vi "PicoScope5000aSettings.vi"(0 "error in":errorcluster, 1 "Channel A Settings":T3={"Enabled"=FALSE, "Coupling"=1, "Range"=6, "Analogue Offset"=0.0, "Bandwidth Limit"=0} {"Bandwidth Limit" items=["Full", "20MHz"]; "Range" items=["10 mV", "20 mV", "50 mV", "100 mV", "200 mV", "500 mV", "1 V", "2 V", "5 V", "10 V", "20 V"]; "Coupling" items=["AC", "DC"]}, 2 "Port 0 Settings":T1={"Enabled"=FALSE, "Logic Level"=9830} {"Logic Level" items=["1.5V TTL"=9830, "2.5V CMOS"=16383]}, 3 "Channel B Settings":T3={"Enabled"=FALSE, "Coupling"=1, "Range"=6, "Analogue Offset"=0.0, "Bandwidth Limit"=0} {"Bandwidth Limit" items=["Full", "20MHz"]; "Range" items=["10 mV", "20 mV", "50 mV", "100 mV", "200 mV", "500 mV", "1 V", "2 V", "5 V", "10 V", "20 V"]; "Coupling" items=["AC", "DC"]}, 5 "handle in":i16, 9 "Device Info":T2, 11 "Trigger Settings":T4={"Trigger Enabled"=FALSE, "Trigger Source"=enum."Channel A", "Trigger Threshold (volts)"=0.0, "Trigger Direction"=2, "Trigger Delay (samples)"=0, "Auto Trigger Time (ms)"=1000} {"Trigger Direction" items=["Rising"=2, "Falling"=3]}, 12 "Channel C Settings":T3={"Enabled"=FALSE, "Coupling"=1, "Range"=6, "Analogue Offset"=0.0, "Bandwidth Limit"=0} {"Bandwidth Limit" items=["Full", "20MHz"]; "Range" items=["10 mV", "20 mV", "50 mV", "100 mV", "200 mV", "500 mV", "1 V", "2 V", "5 V", "10 V", "20 V"]; "Coupling" items=["AC", "DC"]}, 13 "Port 1 Settings":T1={"Enabled"=FALSE, "Logic Level"=9830} {"Logic Level" items=["1.5V TTL"=9830, "2.5V CMOS"=16383]}, 14 "Channel D Settings":T3={"Enabled"=FALSE, "Coupling"=1, "Range"=6, "Analogue Offset"=0.0, "Bandwidth Limit"=0} {"Bandwidth Limit" items=["Full", "20MHz"]; "Range" items=["10 mV", "20 mV", "50 mV", "100 mV", "200 mV", "500 mV", "1 V", "2 V", "5 V", "10 V", "20 V"]; "Coupling" items=["AC", "DC"]}, 15 "Max ADC value":i16) -> (4 "error out":errorcluster, 6 "handle out":i16, 8 "enabled array":i16[](array[numeric]))   [LabVIEW 2010]
doc: "This VI is used to set up the oscilloscope. The inputs are clusters for setting channel and simple trigger settings. Advanced triggers can be set up using PicoScope3000aAdvancedTriggerSettings.vi"
uses:
  ps5000a.dll
  PicoScope5000aAnalogChannelSettings.ctl
  PicoScope5000aDigitalChannelSettings.ctl
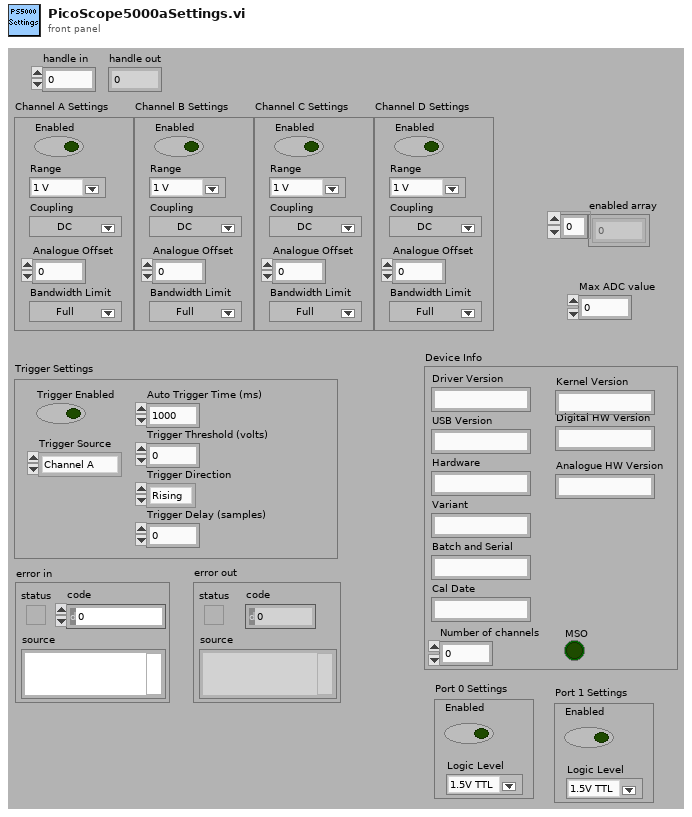
[diagram p1: front panel]
types:
  T1 = typedef "PicoScope5000aDigitalChannelSettings.ctl" = cluster{"Enabled":bool, "Logic Level":i16}
  T2 = cluster{"Driver Version":string, "USB Version":string, "Hardware":string, "Variant":string, "Batch and Serial":string, "Cal Date":string, "Kernel Version":string, "Digital HW Version":string, "Analogue HW Version":string, "MSO":bool, "Number of channels":i16}
  T3 = typedef "PicoScope5000aAnalogChannelSettings.ctl" = cluster{"Enabled":bool, "Coupling":i16, "Range":u16, "Analogue Offset":sgl, "Bandwidth Limit":u32}
  T4 = cluster{"Trigger Enabled":bool, "Trigger Source":enum16{"Channel A", "Channel B", "Channel C", "Channel D", "Ext."}, "Trigger Threshold (volts)":dbl, "Trigger Direction":u16, "Trigger Delay (samples)":u32, "Auto Trigger Time (ms)":i16}
  T5 = enum16{"Channel A", "Channel B", "Channel C", "Channel D", "Ext."}
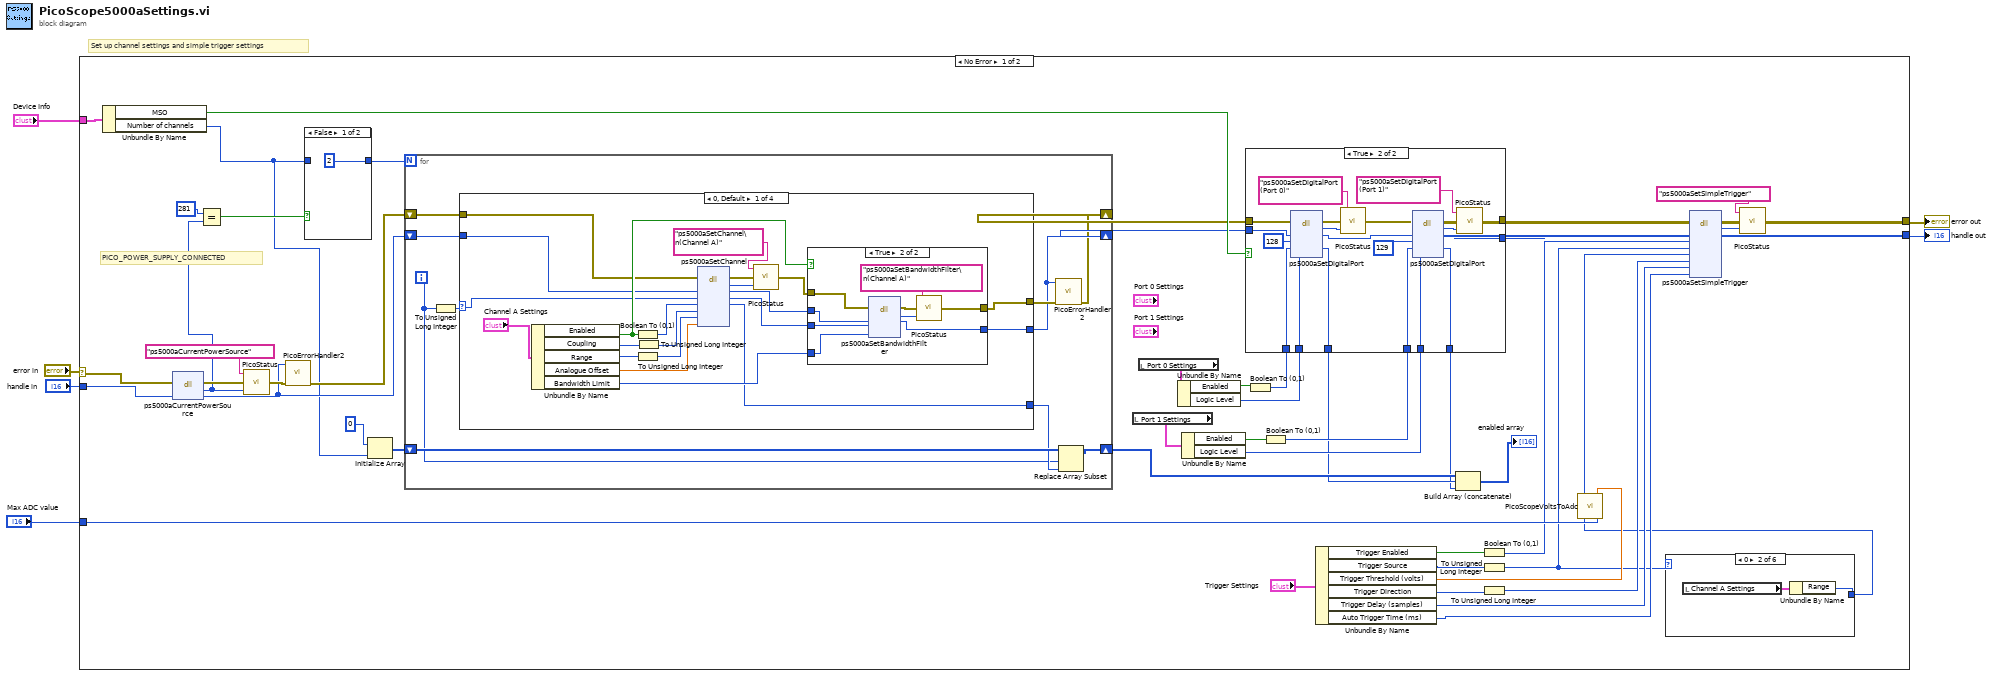
[diagram p0: block diagram]
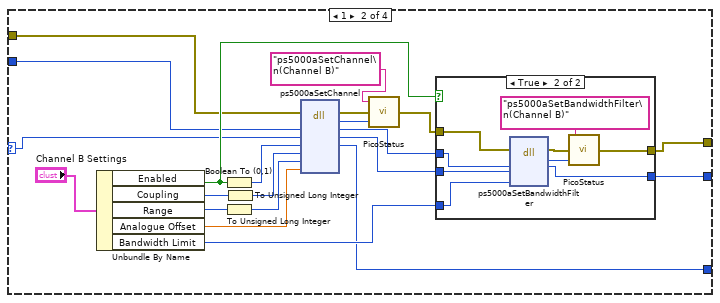
[diagram p4: hidden frame]
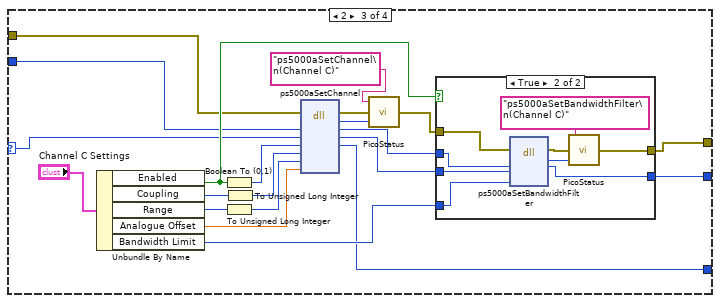
[diagram p6: hidden frame]
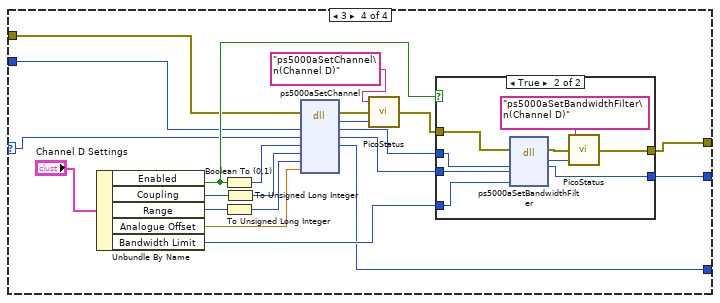
[diagram p8: hidden frame]
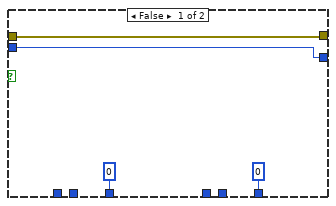
[diagram p10: hidden frame]
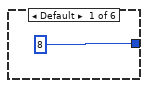
[diagram p11: hidden frame]
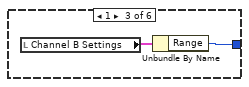
[diagram p12: hidden frame]
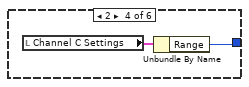
[diagram p13: hidden frame]
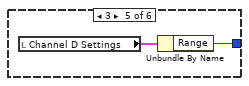
[diagram p14: hidden frame]
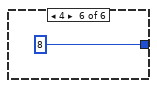
[diagram p15: hidden frame]
diagram:
  # "Set up channel settings and simple trigger settings"
  n1 = case shown="No Error" "error in" {
    selector: "error in" -> [w19 w232]
    tunnel: "handle in" -> [w18 w231]
    tunnel: [w47 w231] -> w4
    tunnel: [w36 w232] -> w3
    tunnel: "Device Info" -> [w42 _]
    tunnel: "Max ADC value" -> [w39 _]
    frame No Error {
      # "PICO_POWER_SUPPLY_CONNECTED"
      n2 = Unbundle By Name(w42) -> ("MSO"=w24:bool, "Number of channels"=w7:i16)
      n3 = dll-call lib="ps5000a.dll" fn="ps5000aCurrentPowerSource"(error in=w19, "handle"=w18) -> (error out=w45:errorcluster, "PICO_STATUS"=w43:u32, "handle"=w16:i16)  [unwired: 2 in, 1 out]
      n4 = Equal?(x=u32 281, y=w43) -> (x = y?=w14:bool)
      n5 = call "PicoStatus.vi"("PICO STATUS"=w43, "error in"=w45, "source"="ps5000aCurrentPowerSource") -> ("error out"=w17:errorcluster)
      n6 = call "PicoErrorHandler2.vi"("error in (no error)"=w17, "handle In"=w16) -> ("error out"=w15:errorcluster)  [unwired: 9 in]
      n7 = case shown="False" w14 {
        tunnel: [2 ("Number of channels") w58] -> w8
        tunnel: w7 -> [_ w58]
        frame False {
        }
        frame True {
        }
      }
      n8 = Initialize Array(i16 0 ("element"), w7) -> (w22:i16[])
      n9 = for {
        N: w8 -> [_]
        shift-right: [w66] -> w12
        shift-left: w22 -> [w68]
        shift-right: [w63] -> w21
        shift-left: w15 -> [w65]
        shift-right: [w61] -> w20
        shift-left: w16 -> [w64]
        i -> [w59]
        n10 = To Unsigned Long Integer(number=w59) -> (unsigned 32bit integer=w60:u32)
        n11 = case shown="0, Default" w60 {
          selector: w60 -> [w69 w101 w133 w165]
          tunnel: [w74 w107 w139 w171] -> w67
          tunnel: w65 -> [w73 w105 w137 w169]
          tunnel: w64 -> [w72 w104 w136 w168]
          tunnel: [w71 w103 w135 w167] -> w62
          tunnel: [w70 w102 w134 w166] -> w61
          frame 0, Default {
            n12 = Unbundle By Name("Channel A Settings") -> ("Enabled"=w78:bool, "Coupling"=w88:i16, "Range"=w89:u16, "Analogue Offset"=w86:sgl, "Bandwidth Limit"=w79:u32)
            n13 = Boolean To (0,1)(Boolean=w78) -> (0, 1=w81:i16)
            n14 = To Unsigned Long Integer(number=w89) -> (unsigned 32bit integer=w85:u32)
            n15 = To Unsigned Long Integer(number=w88) -> (unsigned 32bit integer=w87:u32)
            n16 = dll-call lib="ps5000a.dll" fn="ps5000aSetChannel" ("ps3000.dll:_ps3000_open_unit@0")(error in=w73, "handle"=w72, "channel"=w69, "enabled"=w81, "dc"=w87, "range"=w85, "analogueOffset"=w86) -> (error out=w84:errorcluster, "PICO_STATUS"=w83:u32, "handle"=w76:i16, "channel"=w75:u32, "enabled"=w74:i16)  [unwired: 5 in, 1 out]
            n17 = call "PicoStatus.vi"("PICO STATUS"=w83, "error in"=w84, "source"="ps5000aSetChannel\n(Channel A)") -> ("error out"=w77:errorcluster)
            n18 = case shown="True" w78 {
              tunnel: w77 -> [w91 w97]
              tunnel: [w91 w96] -> w71
              tunnel: [w90 w95] -> w70
              tunnel: w75 -> [_ w94]
              tunnel: w76 -> [w90 w93]
              tunnel: w79 -> [_ w92]
              frame False {
              }
              frame True {
                n19 = dll-call lib="ps5000a.dll" fn="ps5000aSetBandwidthFilter" ("ps3000.dll:_ps3000_open_unit@0")(error in=w97, "handle"=w93, "channel"=w94, "Bandwidth Limit"=w92) -> (error out=w99:errorcluster, "PICO_STATUS"=w98:u32, "handle"=w95:i16)  [unwired: 4 in, 1 out]
                n20 = call "PicoStatus.vi"("PICO STATUS"=w98, "error in"=w99, "source"="ps5000aSetBandwidthFilter\n(Channel A)") -> ("error out"=w96:errorcluster)
              }
            }
          }
          frame 1 {
            n21 = Unbundle By Name("Channel B Settings") -> ("Enabled"=w111:bool, "Coupling"=w120:i16, "Range"=w121:u16, "Analogue Offset"=w118:sgl, "Bandwidth Limit"=w112:u32)
            n22 = Boolean To (0,1)(Boolean=w111) -> (0, 1=w114:i16)
            n23 = To Unsigned Long Integer(number=w121) -> (unsigned 32bit integer=w117:u32)
            n24 = To Unsigned Long Integer(number=w120) -> (unsigned 32bit integer=w119:u32)
            n25 = dll-call lib="ps5000a.dll" fn="ps5000aSetChannel" ("ps3000.dll:_ps3000_open_unit@0")(error in=w105, "handle"=w104, "channel"=w101, "enabled"=w114, "dc"=w119, "range"=w117, "analogueOffset"=w118) -> (error out=w116:errorcluster, "PICO_STATUS"=w115:u32, "handle"=w109:i16, "channel"=w108:u32, "enabled"=w107:i16)  [unwired: 5 in, 1 out]
            n26 = call "PicoStatus.vi"("PICO STATUS"=w115, "error in"=w116, "source"="ps5000aSetChannel\n(Channel B)") -> ("error out"=w110:errorcluster)
            n27 = case shown="True" w111 {
              tunnel: w110 -> [w123 w129]
              tunnel: [w123 w128] -> w103
              tunnel: [w122 w127] -> w102
              tunnel: w108 -> [_ w126]
              tunnel: w109 -> [w122 w125]
              tunnel: w112 -> [_ w124]
              frame False {
              }
              frame True {
                n28 = dll-call lib="ps5000a.dll" fn="ps5000aSetBandwidthFilter" ("ps3000.dll:_ps3000_open_unit@0")(error in=w129, "handle"=w125, "channel"=w126, "Bandwidth Limit"=w124) -> (error out=w131:errorcluster, "PICO_STATUS"=w130:u32, "handle"=w127:i16)  [unwired: 4 in, 1 out]
                n29 = call "PicoStatus.vi"("PICO STATUS"=w130, "error in"=w131, "source"="ps5000aSetBandwidthFilter\n(Channel B)") -> ("error out"=w128:errorcluster)
              }
            }
          }
          frame 2 {
            n30 = Unbundle By Name("Channel C Settings") -> ("Enabled"=w143:bool, "Coupling"=w152:i16, "Range"=w153:u16, "Analogue Offset"=w150:sgl, "Bandwidth Limit"=w144:u32)
            n31 = Boolean To (0,1)(Boolean=w143) -> (0, 1=w146:i16)
            n32 = To Unsigned Long Integer(number=w153) -> (unsigned 32bit integer=w149:u32)
            n33 = To Unsigned Long Integer(number=w152) -> (unsigned 32bit integer=w151:u32)
            n34 = dll-call lib="ps5000a.dll" fn="ps5000aSetChannel" ("ps3000.dll:_ps3000_open_unit@0")(error in=w137, "handle"=w136, "channel"=w133, "enabled"=w146, "dc"=w151, "range"=w149, "analogueOffset"=w150) -> (error out=w148:errorcluster, "PICO_STATUS"=w147:u32, "handle"=w141:i16, "channel"=w140:u32, "enabled"=w139:i16)  [unwired: 5 in, 1 out]
            n35 = call "PicoStatus.vi"("PICO STATUS"=w147, "error in"=w148, "source"="ps5000aSetChannel\n(Channel C)") -> ("error out"=w142:errorcluster)
            n36 = case shown="True" w143 {
              tunnel: w142 -> [w155 w161]
              tunnel: [w155 w160] -> w135
              tunnel: [w154 w159] -> w134
              tunnel: w140 -> [_ w158]
              tunnel: w141 -> [w154 w157]
              tunnel: w144 -> [_ w156]
              frame False {
              }
              frame True {
                n37 = dll-call lib="ps5000a.dll" fn="ps5000aSetBandwidthFilter" ("ps3000.dll:_ps3000_open_unit@0")(error in=w161, "handle"=w157, "channel"=w158, "Bandwidth Limit"=w156) -> (error out=w163:errorcluster, "PICO_STATUS"=w162:u32, "handle"=w159:i16)  [unwired: 4 in, 1 out]
                n38 = call "PicoStatus.vi"("PICO STATUS"=w162, "error in"=w163, "source"="ps5000aSetBandwidthFilter\n(Channel C)") -> ("error out"=w160:errorcluster)
              }
            }
          }
          frame 3 {
            n39 = Unbundle By Name("Channel D Settings") -> ("Enabled"=w175:bool, "Coupling"=w184:i16, "Range"=w185:u16, "Analogue Offset"=w182:sgl, "Bandwidth Limit"=w176:u32)
            n40 = Boolean To (0,1)(Boolean=w175) -> (0, 1=w178:i16)
            n41 = To Unsigned Long Integer(number=w185) -> (unsigned 32bit integer=w181:u32)
            n42 = To Unsigned Long Integer(number=w184) -> (unsigned 32bit integer=w183:u32)
            n43 = dll-call lib="ps5000a.dll" fn="ps5000aSetChannel" ("ps3000.dll:_ps3000_open_unit@0")(error in=w169, "handle"=w168, "channel"=w165, "enabled"=w178, "dc"=w183, "range"=w181, "analogueOffset"=w182) -> (error out=w180:errorcluster, "PICO_STATUS"=w179:u32, "handle"=w173:i16, "channel"=w172:u32, "enabled"=w171:i16)  [unwired: 5 in, 1 out]
            n44 = call "PicoStatus.vi"("PICO STATUS"=w179, "error in"=w180, "source"="ps5000aSetChannel\n(Channel D)") -> ("error out"=w174:errorcluster)
            n45 = case shown="True" w175 {
              tunnel: w174 -> [w187 w193]
              tunnel: [w187 w192] -> w167
              tunnel: [w186 w191] -> w166
              tunnel: w172 -> [_ w190]
              tunnel: w173 -> [w186 w189]
              tunnel: w176 -> [_ w188]
              frame False {
              }
              frame True {
                n46 = dll-call lib="ps5000a.dll" fn="ps5000aSetBandwidthFilter" ("ps3000.dll:_ps3000_open_unit@0")(error in=w193, "handle"=w189, "channel"=w190, "Bandwidth Limit"=w188) -> (error out=w195:errorcluster, "PICO_STATUS"=w194:u32, "handle"=w191:i16)  [unwired: 4 in, 1 out]
                n47 = call "PicoStatus.vi"("PICO STATUS"=w194, "error in"=w195, "source"="ps5000aSetBandwidthFilter\n(Channel D)") -> ("error out"=w192:errorcluster)
              }
            }
          }
        }
        n48 = call "PicoErrorHandler2.vi"("error in (no error)"=w62, "handle In"=w61) -> ("error out"=w63:errorcluster)  [unwired: 9 in]
        n49 = Replace Array Subset(array=w68, new element=w67, index=w59) -> (w66:i16[])
      }
      n50 = local read "Port 1 Settings"() -> (w34:T1)
      n51 = local read "Port 0 Settings"() -> (w35:T1)
      n52 = Unbundle By Name(w35) -> ("Enabled"=w33:bool, "Logic Level"=w31:i16)
      n53 = Unbundle By Name(w34) -> ("Enabled"=w30:bool, "Logic Level"=w28:i16)
      n54 = Boolean To (0,1)(Boolean=w33) -> (0, 1=w32:i16)
      n55 = Boolean To (0,1)(Boolean=w30) -> (0, 1=w29:i16)
      n56 = case shown="True" w24 {
        tunnel: [w200 w212] -> w27
        tunnel: w32 -> [_ w209]
        tunnel: w31 -> [_ w208]
        tunnel: w29 -> [_ w207]
        tunnel: w28 -> [_ w206]
        tunnel: w21 -> [w200 w205]
        tunnel: w20 -> [w199 w204]
        tunnel: [w199 w203] -> w26
        tunnel: [i16 0 ("enabled") w202] -> w11
        tunnel: [i16 0 ("enabled") w201] -> w10
        frame False {
        }
        frame True {
          n57 = dll-call lib="PS5000a.dll" fn="ps5000aSetDigitalPort"(error in=w205, "handle"=w204, "port"=u32 128, "enabled"=w209, "logicLevel"=w208) -> (error out=w220:errorcluster, "PICO_STATUS"=w217:u32, "handle"=w213:i16, "enabled"=w202:i16)  [unwired: 4 in, 1 out]
          n58 = call "PicoStatus.vi"("PICO STATUS"=w217, "error in"=w220, "source"="ps5000aSetDigitalPort (Port 0)") -> ("error out"=w214:errorcluster)
          n59 = dll-call lib="PS5000a.dll" fn="ps5000aSetDigitalPort"(error in=w214, "handle"=w213, "port"=u32 129, "enabled"=w207, "logicLevel"=w206) -> (error out=w216:errorcluster, "PICO_STATUS"=w215:u32, "handle"=w203:i16, "enabled"=w201:i16)  [unwired: 4 in, 1 out]
          n60 = call "PicoStatus.vi"("PICO STATUS"=w215, "error in"=w216, "source"="ps5000aSetDigitalPort (Port 1)") -> ("error out"=w212:errorcluster)
        }
      }
      n61 = Unbundle By Name("Trigger Settings") -> ("Trigger Enabled"=w51:bool, "Trigger Source"=w52:T5, "Trigger Threshold (volts)"=w40:dbl, "Trigger Direction"=w54:u16, "Trigger Delay (samples)"=w53:u32, "Auto Trigger Time (ms)"=w38:i16)
      n62 = Build Array (concatenate)(w12, w11, w10) -> (→"enabled array":i16[])
      n63 = Boolean To (0,1)(Boolean=w51) -> (0, 1=w25:i16)
      n64 = To Unsigned Long Integer(number=w52) -> (unsigned 32bit integer=w37:u32)
      n65 = To Unsigned Long Integer(number=w54) -> (unsigned 32bit integer=w56:u32)
      n66 = case shown="0" w37 {
        tunnel: [u16 8 ("Range") w222 w224 w226 w228 u16 8 ("Range")] -> w13
        frame Default {
        }
        frame 0 {
          n67 = local read "Channel A Settings"() -> (w223:T3)
          n68 = Unbundle By Name(w223) -> ("Range"=w222:u16)
        }
        frame 1 {
          n69 = local read "Channel B Settings"() -> (w225:T3)
          n70 = Unbundle By Name(w225) -> ("Range"=w224:u16)
        }
        frame 2 {
          n71 = local read "Channel C Settings"() -> (w227:T3)
          n72 = Unbundle By Name(w227) -> ("Range"=w226:u16)
        }
        frame 3 {
          n73 = local read "Channel D Settings"() -> (w229:T3)
          n74 = Unbundle By Name(w229) -> ("Range"=w228:u16)
        }
        frame 4 {
        }
      }
      n75 = call "PicoScopeVoltsToAdc.vi"("Max_adc"=w39, "Units"=w40, "Range Index"=w13) -> ("ADC count"=w41:i16)
      n76 = dll-call lib="ps5000a.dll" fn="ps5000aSetSimpleTrigger" ("ps3000.dll:_ps3000_open_unit@0")(error in=w27, "handle"=w26, "enable"=w25, "source"=w37, "threshold"=w41, "direction"=w56, "delay"=w53, "autoTrigger_ms"=w38) -> (error out=w49:errorcluster, "PICO_STATUS"=w50:u32, "handle"=w47:i16)  [unwired: 8 in, 1 out]
      n77 = call "PicoStatus.vi"("PICO STATUS"=w50, "error in"=w49, "source"="ps5000aSetSimpleTrigger") -> ("error out"=w36:errorcluster)
    }
    frame Error {
    }
  }
  "handle out" <- w4
  "error out" <- w3
